vi "Parse Request.vi"(8 "error in (no error)":errorcluster, 10 "<JSON> Requests":string) -> (0 "error out":errorcluster, 1 "Params":string, 2 "Methods":string, 4 "IDs":string)   [LabVIEW 2019, in "JSON-RPC.lvlib"]
doc: "Parse a Request object to extract an object's <b>method</b>, <b>params</b>, and <b>id</b>.\n\nThe <b>params</b> datatype is a JSON object and will need further processing to convert to LabVIEW data.\n\nhttps://www.jsonrpc.org/specification"
uses:
  JSON-RPC.lvlib
  private/Parse Request-JSONtext.vi/66b5d778-a0b8-403e-b727-bb36a32d382a.vi
  private/Parse Request-JSONtext.vi/6814ee06-2257-4c2f-8f04-31d91309bef7.vi
  private/Parse Request-JSONtext.vi/f1c5ac56-d3e8-467f-aff4-e25fa4ac2541.vi
  <vilib>/JDP Science/JSONtext/Get all Object Items.vi
  <vilib>/JDP Science/JSONtext/JSON text to Variant.vi
  <vilib>/JDP Science/JSONtext/LVClass Serializer/JSONtext LVClass Serializer.lvclass
  <vilib>/JDP Science/JSONtext/JSONtext.lvlib
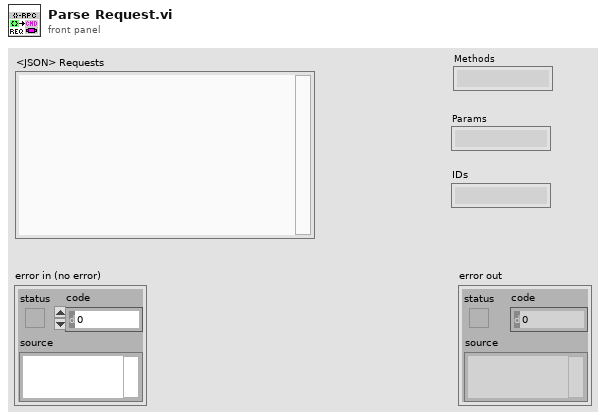
[diagram p1: front panel]
types:
  T1 = enum16{"Parse Error", "Invalid Request", "Method not found", "Invalid params", "Internal error", "Server error"}
  T2 = typedef "JSONtext.lvlib/JSON Value Type.ctl" = enum16{"Not a JSON Value", "JSON Object", "JSON Array", "String", "Number", "true", "false", "null"}
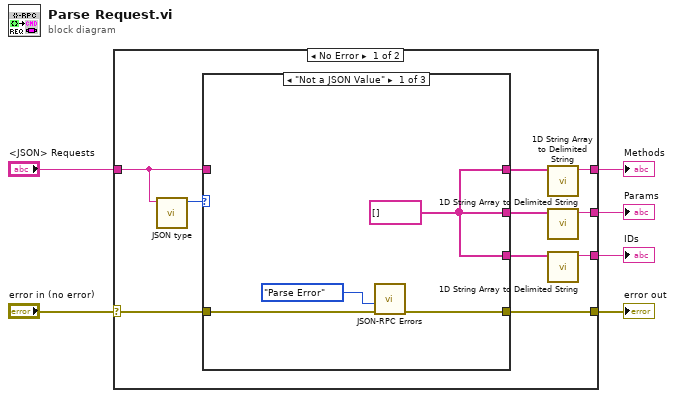
[diagram p0: block diagram]
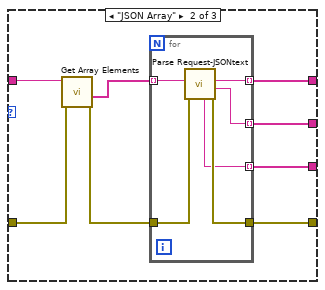
[diagram p2: hidden frame]
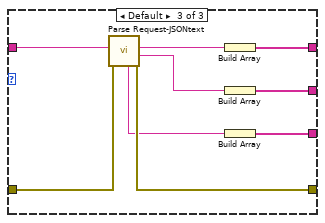
[diagram p3: hidden frame]
diagram:
  n1 = case shown="No Error" "error in (no error)" {
    selector: "error in (no error)" -> [w15 w44]
    tunnel: [w7 w44] -> w5
    tunnel: "<JSON> Requests" -> [w14 _]
    tunnel: [w12 _] -> w2
    tunnel: [w13 _] -> w3
    tunnel: [w11 _] -> w1
    frame No Error {
      n2 = call <vilib>:"JSON type.vi"("JSON"=w14) -> ("JSON Value Type"=w16:T2)  [unwired: 9 in, 1 out]
      n3 = case shown="\"Not a JSON Value\"" w16 {
        tunnel: w15 -> [w18 w24 w42]
        tunnel: [w19 w28 w41] -> w7
        tunnel: w14 -> [_ w25 w43]
        tunnel: [w20 w27 w35] -> w10
        tunnel: [w20 w26 w37] -> w8
        tunnel: [w20 w23 w39] -> w9
        frame "Not a JSON Value" {
          w20 = string[] []
          n4 = call "JSON-RPC Errors.vi"("error in"=w18, "Enum"=T1."Parse Error") -> ("error out"=w19:errorcluster)  [unwired: 9 in]
        }
        frame "JSON Array" {
          n5 = call <vilib>:"Get Array Elements.vi"("error in (no error)"=w24, "JSON"=w25) -> ("error out"=w21:errorcluster, "<JSON>"=w22:string[])  [unwired: 7 in, 1 out]
          n6 = for {
            tunnel: w22 -> [w32] mode=indexing
            tunnel: [w31] -> w27 mode=indexing
            tunnel: [w29] -> w26 mode=indexing
            tunnel: [w30] -> w23 mode=indexing
            tunnel: w21 -> [w33]
            tunnel: [w34] -> w28
            n7 = call "Parse Request-JSONtext.vi"("error in (no error)"=w33, "<JSON> Request"=w32) -> ("error out"=w34:errorcluster, "params"=w29:string, "method"=w31:string, "id"=w30:string)  [unwired: 6 in]
          }
        }
        frame Default {
          n8 = call "Parse Request-JSONtext.vi"("error in (no error)"=w42, "<JSON> Request"=w43) -> ("error out"=w41:errorcluster, "params"=w38:string, "method"=w36:string, "id"=w40:string)  [unwired: 6 in]
          n9 = Build Array(w36) -> (w35:string[])
          n10 = Build Array(w38) -> (w37:string[])
          n11 = Build Array(w40) -> (w39:string[])
        }
      }
      n12 = call <vilib>:"1D String Array to Delimited String.vi"("string array"=w10) -> ("delimited string"=w13:string)  [unwired: 10 in]
      n13 = call <vilib>:"1D String Array to Delimited String.vi"("string array"=w8) -> ("delimited string"=w12:string)  [unwired: 10 in]
      n14 = call <vilib>:"1D String Array to Delimited String.vi"("string array"=w9) -> ("delimited string"=w11:string)  [unwired: 10 in]
    }
    frame Error {
    }
  }
  "error out" <- w5
  "Methods" <- w3
  "Params" <- w2
  "IDs" <- w1
